vi "file_path.vi"(9 "string":string, 10 "number":i32, 11 "Data Directory":path) -> (2 "path":path)   [LabVIEW 2026]
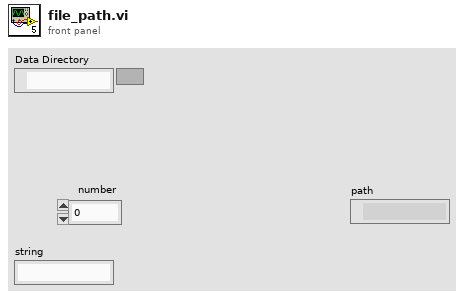
[diagram p1: front panel]
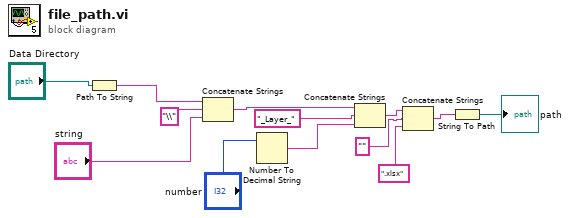
[diagram p0: block diagram]
diagram:
  n1 = Path To String(path="Data Directory") -> (string=w12:string)
  n2 = Concatenate Strings(w12, "\\" ("string"), "string") -> (w9:string)
  n3 = Number To Decimal String(number="number") -> (decimal integer string=w6:string)  [unwired: 1 in]
  n4 = Concatenate Strings(w9, "_Layer_" ("string"), w6) -> (w5:string)
  n5 = Concatenate Strings(w5, "" ("string"), ".xlsx" ("string")) -> (w4:string)
  n6 = String To Path(string=w4) -> (path=→"path":path)
